vi "Plot MAX Setting.vi"(8 "min":dbl=-0.175 format="%#_13g", 9 "bin length":dbl=0.05 format="%#_13g", 11 "MAX":dbl) -> (0 "New MAX":dbl, 1 "New MIN":dbl, 3 "New bin":dbl)   [LabVIEW 2018]
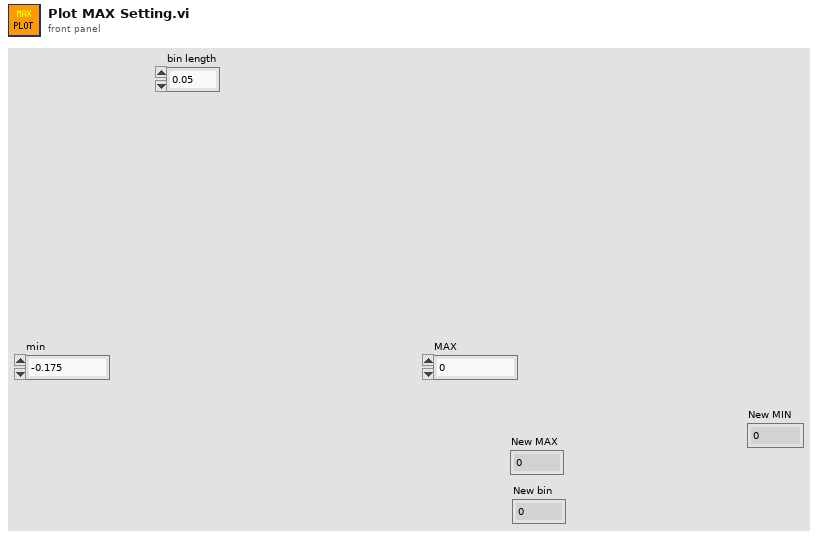
[diagram p1: front panel]
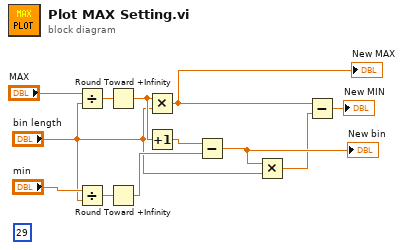
[diagram p0: block diagram]
diagram:
  (unwired) 29 ("# bins")
  n1 = Divide(x="MAX", y="bin length") -> (x/y=w12:dbl)
  n2 = Divide(x="min", y="bin length") -> (x/y=w10:dbl)
  n3 = Round Toward +Infinity(x=w12) -> (ceil(x): smallest int >= x=w11:dbl)
  n4 = Round Toward +Infinity(x=w10) -> (ceil(x): smallest int >= x=w7:dbl)
  n5 = Multiply(x=w11, y="bin length") -> (x*y=w3:dbl)
  "New MAX" <- w3
  n6 = Increment(x=w11) -> (x+1=w8:dbl)
  n7 = Subtract(x=w8, y=w7) -> (x-y=w5:dbl)
  "New bin" <- w5
  n8 = Multiply(x=w5, y="bin length") -> (x*y=w2:dbl)
  n9 = Subtract(x=w3, y=w2) -> (x-y=→"New MIN":dbl)
